vi "Express VI - Filter.vi"() -> ()   [LabVIEW 2020]
doc: "This example shows some results of the use of the Filter Express VI."
uses:
  Instance           2 14Saved   Filter .vi
  <vilib>/express/express analysis/Spectral/Block/exnSpectralBlock spectral measurements PSD poly.vi
  <vilib>/express/express analysis/Spectral/Block/exnSpectralBlock spectral measurements PSD DDT.vi
  <vilib>/express/express analysis/Spectral/XNode/ExpressSpectralMeasurementsBlockNode.xnode
panel:
  out "Sine waveform":dynamicdata(graph)
  in  "fc":dbl=50.0 caption="Lower Cut-Off"
  in  "fc":dbl=100.0 caption="Lower Cut-Off"
  in  "Frequency 2":dbl(slide)=489.0 scale=1.0..5000.0
  out "PSD":dynamicdata(graph)
  out "Highpass Results":dynamicdata(graph)
  out "Lowpass Results":dynamicdata(graph)
  in  "Frequency":dbl(slide)=489.0 scale=1.0..5000.0
  in  "Stop":bool
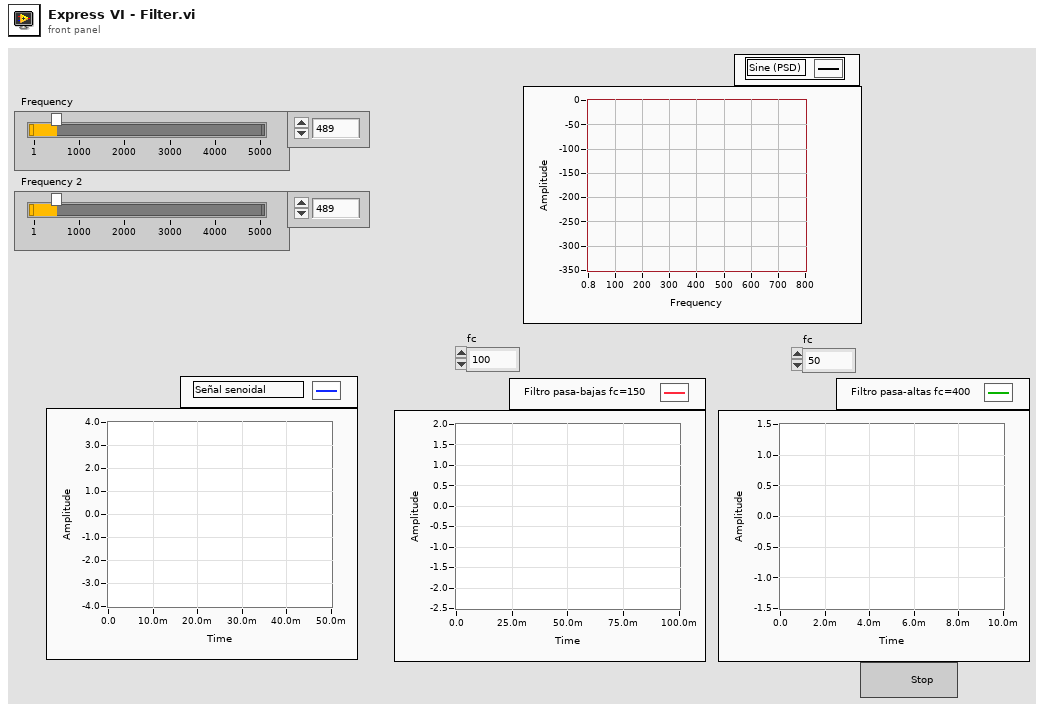
[diagram p1: front panel]
types:
  T1 = cluster{"averaging mode":u16, "weighting mode":u16, "number of averages":u32}
  T2 = cluster{"dB On (F)":bool, "unwrap phase (F)":bool, "convert to degree (F)":bool}
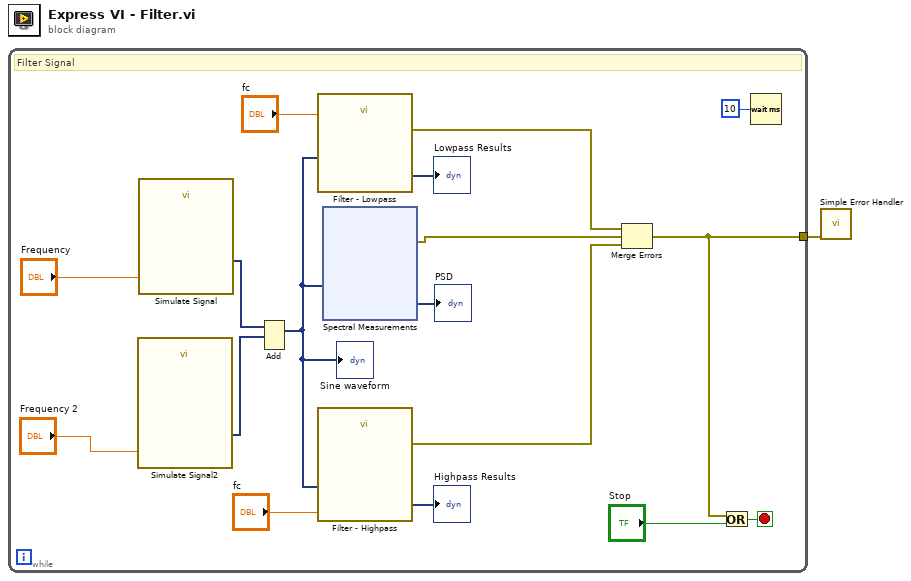
[diagram p0: block diagram]
diagram:
  n1 = while {
    tunnel: [w10] -> w1
    stop <- w11 stop-if-true
    # "Filter Signal"
    n2 = call "Simulate Signal2"("Frequency"="Frequency 2") -> ("Sine"=w5:dynamicdata)  [unwired: 13 in, 1 out]
    n3 = call "Simulate Signal"("Frequency"="Frequency") -> ("Sine"=w6:dynamicdata)  [unwired: 13 in, 1 out]
    n4 = Add(1:w5, 2:w6) -> (0:w2:dynamicdata)  [unwired: 1 in, 1 out]
    "Sine waveform" <- w2
    n5 = call "Filter - Lowpass"("Lower Cut-Off"="fc", "Signal"=w2) -> ("error out"=w13:errorcluster, "Filtered Signal"=→"Lowpass Results":dynamicdata)  [unwired: 8 in]
    n6 = call "Filter - Highpass"("Lower Cut-Off"="fc", "Signal"=w2) -> ("error out"=w12:errorcluster, "Filtered Signal"=→"Highpass Results":dynamicdata)  [unwired: 8 in]
    n7 = xnode "Spectral Measurements"("Signals"=w2) -> ("PSD"=→"PSD":dynamicdata, "error out"=w8:errorcluster)  [unwired: 1 in]
    n8 = Merge Errors(w13, w8, w12) -> (w10:errorcluster)
    n9 = Or(x=w10, y="Stop") -> (x .or. y?=w11:bool)
    n10 = Wait (ms)(milliseconds to wait=u32 10) -> ()  [unwired: 1 out]
  }
  n11 = call <vilib>:"Simple Error Handler.vi"("error in (no error)"=w1) -> ()  [unwired: 4 in, 5 out]
